vi "List VIs without Test Coverage.vi"(8 "error in (no error)":errorcluster, 9 "Tests Root":path, 10 "Source Root":path) -> (0 "error out":errorcluster, 1 "Test VIs":path[](array[path]), 2 "VIs without test coverage":string[](array[string]))   [LabVIEW 2020]
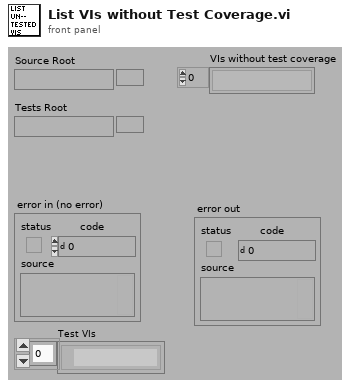
[diagram p1: front panel]
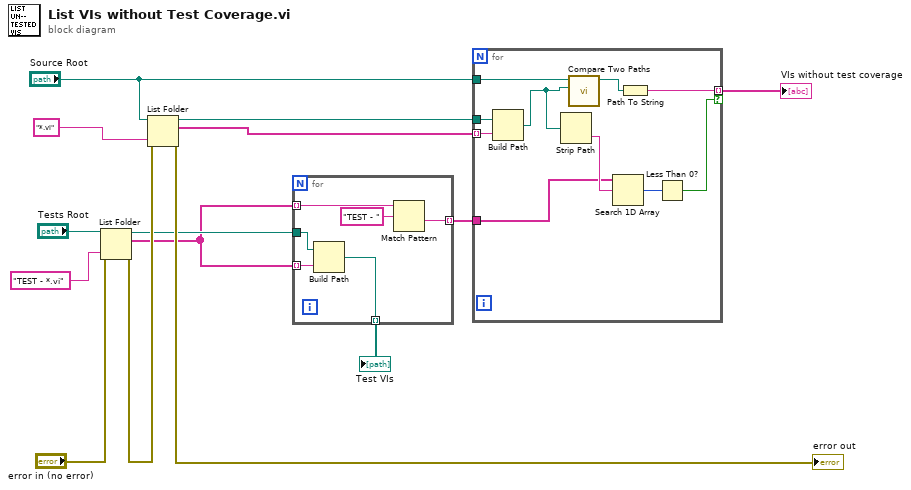
[diagram p0: block diagram]
diagram:
  n1 = List Folder(path="Tests Root", pattern="TEST - *.vi", error in="error in (no error)") -> (path out=w3:path, filenames=w2:string[], error out=w10:errorcluster)  [unwired: 1 in, 1 out]
  n2 = List Folder(path="Source Root", pattern="*.vi", error in=w10) -> (path out=w5:path, filenames=w4:string[], error out=→"error out":errorcluster)  [unwired: 1 in, 1 out]
  n3 = for {
    tunnel: w2 -> [w20] mode=indexing
    tunnel: [w18] -> w9 mode=indexing
    tunnel: w3 -> [w17]
    tunnel: w2 -> [w16] mode=indexing
    tunnel: [w15] -> w1 mode=indexing
    n4 = Build Path(base path=w17, name or relative path=w16) -> (appended path=w15:path)
    n5 = Match Pattern(string=w20, regular expression="TEST - ") -> (after substring=w18:string)  [unwired: 1 in, 3 out]
  }
  "Test VIs" <- w1
  n6 = for {
    tunnel: w9 -> [w29]
    tunnel: "Source Root" -> [w22]
    tunnel: [w27] -> w14 mode=indexing if=w24
    tunnel: w5 -> [w26]
    tunnel: w4 -> [w25] mode=indexing
    n7 = Build Path(base path=w26, name or relative path=w25) -> (appended path=w21:path)
    n8 = Strip Path(path=w21) -> (name=w30:string)  [unwired: 1 out]
    n9 = call <vilib>:"Compare Two Paths.vi"("Path 2"=w21, "Path 1"=w22) -> ("Relative Path from 1 to 2"=w23:path)  [unwired: 6 in, 3 out]
    n10 = Search 1D Array(1D array=w29, element=w30) -> (index of element=w28:i32)  [unwired: 1 in]
    n11 = Path To String(path=w23) -> (string=w27:string)
    n12 = Less Than 0?(x=w28) -> (x < 0?=w24:bool)
  }
  "VIs without test coverage" <- w14
